vi "set OBW - RBW or VBW.vi"(6 "BW Auto?":bool, 8 "error in (no error)":errorcluster, 9 "BW Type":T1, 10 "BW Value (Hz)":dbl format="%#_6p", 11 "FSV-40N in":refnum<class "FSV-40N.lvclass">) -> (0 "error out":errorcluster, 3 "FSV-40N out":refnum<class "FSV-40N.lvclass">)   [LabVIEW 2023, in "Spectrum Analyzer.lvlib" / "FSV-40N.lvclass"]
uses:
  FSV-40N.lvclass
  FSV-40N.lvclass/FSV-40N.ctl
  TYPE DEFINITION/TYPE RBW and VBW Select.ctl
  Spectrum Analyzer.lvlib
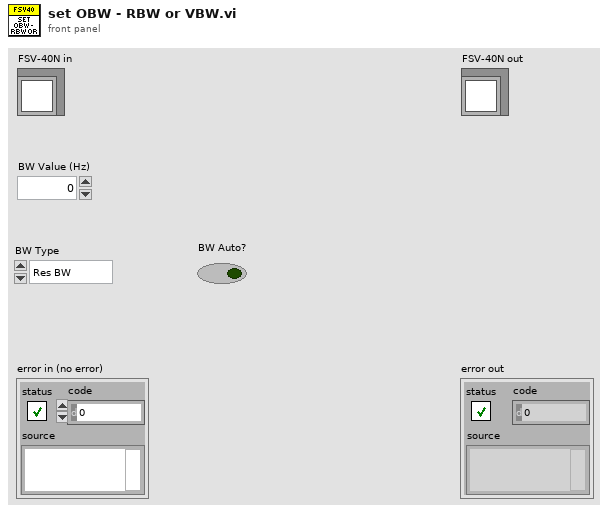
[diagram p1: front panel]
types:
  T1 = typedef "Spectrum Analyzer.lvlib/TYPE RBW and VBW Select.ctl" = enum16{"Res BW", "Video BW"}
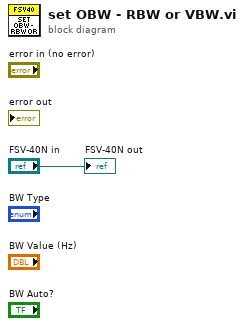
[diagram p0: block diagram]
diagram:
  "FSV-40N out" <- "FSV-40N in"
